vi "XY Sample Stage Mark Points Holder.vi"(2 "Actions":T1=enum."Read", 7 "(X, Y) Points":dbl[](array[numeric])) -> (4 "Marked Points":cluster{dbl[], dbl[]})   [LabVIEW 2016]
uses:
  XY Sample Stage Controls/XY Sample Stage History Actions.ctl
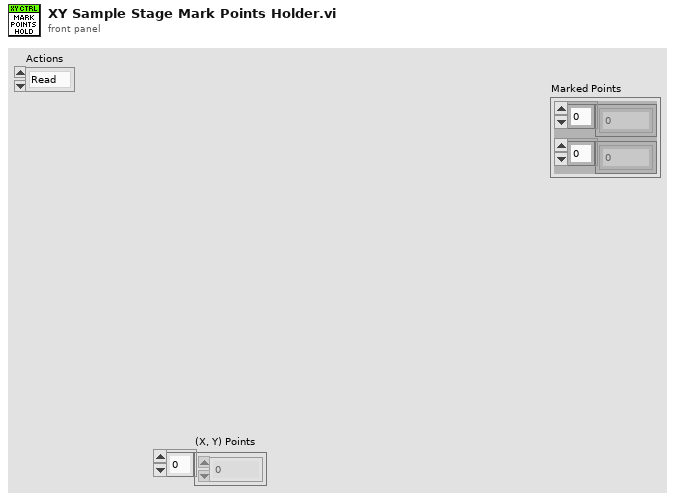
[diagram p1: front panel]
types:
  T1 = typedef "XY Sample Stage History Actions.ctl" = enum16{"Reset", "Write", "Read", "Set Zero"}
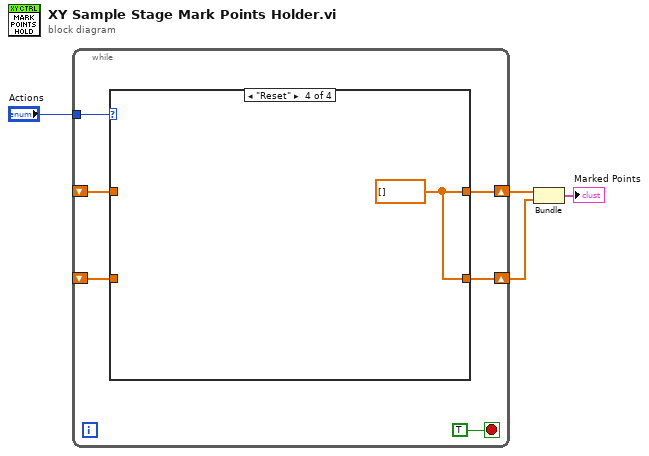
[diagram p0: block diagram]
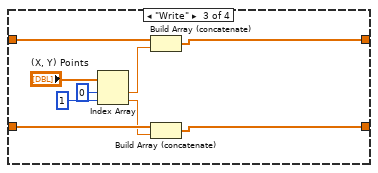
[diagram p4: hidden frame]
diagram:
  n1 = while {
    shift-right: [w8] -> w2
    shift-left: _ -> [w6]
    shift-right: [w7] -> w1
    shift-left: _ -> [w5]
    tunnel: "Actions" -> [w9]
    stop <- TRUE stop-if-true
    n2 = case shown="\"Reset\"" w9 {
      tunnel: [w12 w14 w16 w24] -> w8
      tunnel: [w11 w13 w15 w24] -> w7
      tunnel: w6 -> [w12 w14 w23 _]
      tunnel: w5 -> [w11 w13 w22 _]
      frame "Read", Default {
      }
      frame "Set Zero" {
      }
      frame "Write" {
        n3 = Index Array(array="(X, Y) Points", index #1=0 ("index"), index #2=1 ("index")) -> (element #1=w18:dbl, element #2=w17:dbl)
        n4 = Build Array (concatenate)(w23, w18) -> (w16:dbl[])
        n5 = Build Array (concatenate)(w22, w17) -> (w15:dbl[])
      }
      frame "Reset" {
        w24 = dbl[] []
      }
    }
  }
  n6 = Bundle(w2, w1) -> (→"Marked Points":cluster{dbl[], dbl[]})  [unwired: 1 in]
